vi "Untitled 3.vi"   [LabVIEW 2023]
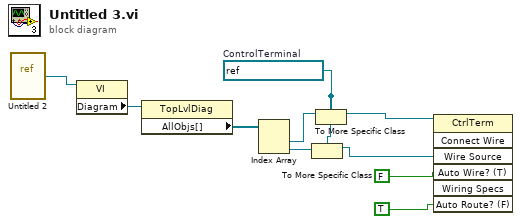
[diagram p0: block diagram]
diagram:
  w5 = refnum<vi> refnum  # ControlTerminal
  n1 = vi-ref "Untitled 2.vi"() -> (w10:refnum<vi>)
  n2 = property class="VI"(reference=w10) -> ("Diagram"=w9:refnum<vi>)  [unwired: 1 in, 2 out]
  n3 = property class="TopLvlDiag"(reference=w9) -> ("AllObjs[]"=w8:refnum<vi>[])  [unwired: 1 in, 2 out]
  n4 = Index Array(array=w8) -> (element #1=w6:refnum<vi>, element #2=w7:refnum<vi>)  [unwired: 2 in]
  n5 = To More Specific Class(target class=w5, reference=w7) -> (specific class reference=w3:refnum<vi>)  [unwired: 1 in, 1 out]
  n6 = To More Specific Class(target class=w5, reference=w6) -> (specific class reference=w4:refnum<vi>)  [unwired: 1 in, 1 out]
  n7 = invoke class="CtrlTerm" method="Connect Wire"(reference=w4, "Wire Source"=w3, "Auto Wire? (T)"=FALSE, "Auto Route? (F)"=TRUE) -> ()  [unwired: 3 in, 7 out]
